vi "HandShaking.vi"(6 "Elapsed Time":u32, 8 "error in":errorcluster, 9 "Sequence Context":refnum<k7>, 10 "Stop":refnum<user-event>, 11 "PreUUT":refnum<class "PreUUT.lvclass">=refnum) -> (0 "error out":errorcluster, 3 "PreUUT out":refnum<class "PreUUT.lvclass">)   [LabVIEW 2025, in "PreUUT.lvclass"]
uses:
  PreUUT.lvclass
  C:/Working copy/TS Manager/Plugin/Tests/Submodule EOL/TS Execution Interface/OPC UA/Abstract.lvclass
  OPC UA/Tester Tx Dataset.ctl
  8b7150cd-7e9f-4590-a01f-0e8ee575d47c.vi
  OPC UA/Read Tx to PLC.vi
  OPC UA/Read Rx from PLC.vi
  OPC UA/Abstract.lvclass
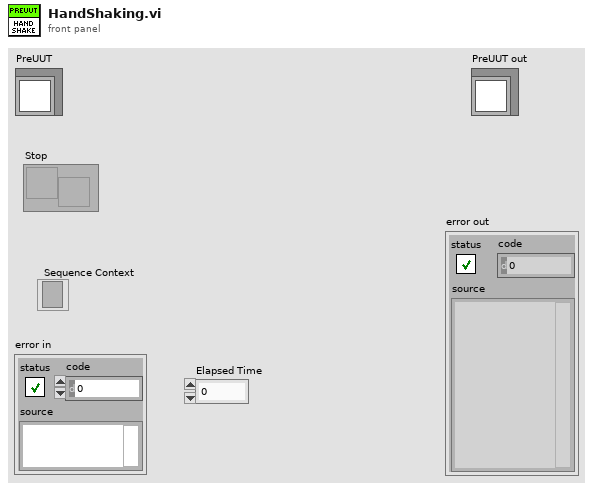
[diagram p1: front panel]
types:
  T1 = typedef "Abstract.lvclass/Tester Tx Dataset.ctl" = cluster{"Fault":bool, "StepNo":u32, "Ready":bool, "HighVoltage":bool, "TestRunning":bool, "ResultsReady":bool, "Results":u32, "ElapsedTime":u32, "Online":bool, "TimeCompleted":i32[], "Timeout":bool, "Heartbeat":bool}
  T2 = typedef "OPC UA.lvlib/OPC UA.lvclass/Tester Rx Dataset.ctl" = cluster{"Start":bool, "NestStatus":bool, "PalletID":u32, "BarcodeData":string, "StepEcho":u32, "Cylinder_1":bool, "Cylinder_2":bool, "Cylinder_3":bool, "Cylinder_4":bool, "Cylinder_5":bool, "ResultsAck":bool, "Reset":bool, "Stop":bool, "FaultCode":u32}
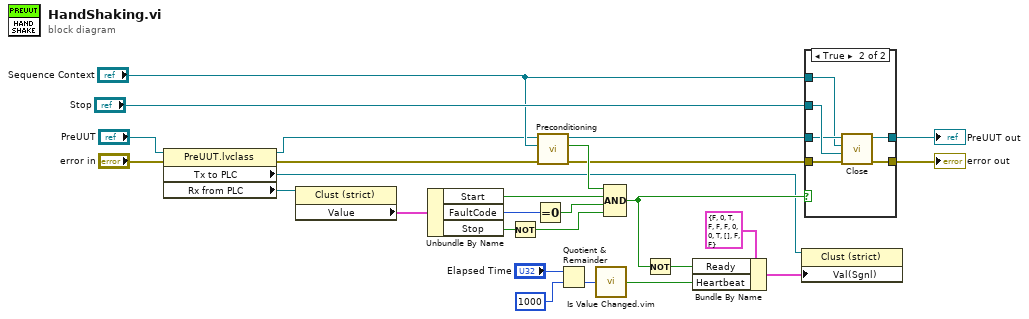
[diagram p0: block diagram]
diagram:
  n1 = property class="PreUUT.lvclass"(reference="PreUUT", error in="error in") -> (reference out=w7:refnum<class "PreUUT.lvclass">, error out=w5:errorcluster, "Tx to PLC"=w1:refnum<vi>, "Rx from PLC"=w2:refnum<vi>)
  n2 = property class="Clust (strict)"(reference=w2) -> ("Value"=w4:T2)  [unwired: 1 in, 2 out]
  n3 = Unbundle By Name(w4) -> ("Start"=w21:bool, "FaultCode"=w23:u32, "Stop"=w24:bool)
  n4 = Not(x=w24) -> (.not. x?=w25:bool)
  n5 = Equal To 0?(x=w23) -> (x = 0?=w22:bool)
  n6 = call "Preconditioning.vi"("error in"=w5, "Sequence Context"="Sequence Context", "PreUUT"=w7) -> ("error out"=w3:errorcluster, "Preconditioning"=w9:bool, "PreUUT out"=w13:refnum<class "PreUUT.lvclass">)  [unwired: 6 in]
  n7 = Quotient & Remainder(x="Elapsed Time", y=u32 1000) -> (floor(x/y)=w17:u32)  [unwired: 1 out]
  n8 = call "Is Value Changed.vim"("value"=w17) -> ("changed or first call?"=w16:bool)
  n9 = Compound Arithmetic op=AND(w9, w21, w22, w25) -> (w11:bool)
  n10 = Not(x=w11) -> (.not. x?=w15:bool)
  n11 = Bundle By Name(cluster=T1 {"Fault"=FALSE, "StepNo"=0, "Ready"=TRUE, "HighVoltage"=FALSE, "TestRunning"=FALSE, "ResultsReady"=FALSE, "Results"=0, "ElapsedTime"=0, "Online"=TRUE, "TimeCompleted"=[], "Timeout"=FALSE, "Heartbeat"=FALSE} ("Value"), "Ready"=w15, "Heartbeat"=w16) -> (w20:T1)
  n12 = property class="Clust (strict)"(reference=w1, "Val(Sgnl)"=w20) -> ()  [unwired: 1 in, 2 out]
  n13 = case shown="True" w11 {
    tunnel: "Stop" -> [_ w33]
    tunnel: w3 -> [w28 w35]
    tunnel: [w28 w34] -> w27
    tunnel: w13 -> [w29 w32]
    tunnel: [w29 w31] -> w26
    tunnel: "Sequence Context" -> [_ w30]
    frame False {
    }
    frame True {
      n14 = call-dynamic "Close.vi"("error in (no error)"=w35, "Stop Event"=w33, "Sequence Context"=w30, "Abstract"=w32) -> ("error out"=w34:errorcluster, "Abstract out"=w31:refnum<class "PreUUT.lvclass">)  [unwired: 6 in]
    }
  }
  "error out" <- w27
  "PreUUT out" <- w26
